vi "AuthService StartLogin.vi"(6 "contextId":T1, 8 "error in":errorcluster, 9 "timeout (ms)":i32=-1, 10 "Request Data":T3, 11 "gRPC ID":T1) -> (0 "error out":errorcluster, 2 "Response Data":T2, 3 "gRPC ID out":T1)   [LabVIEW 2020, in "grpc-auth_client.lvlib"]
uses:
  grpc-auth_client.lvlib
  <vilib>/gRPC/LabVIEW gRPC Library/Shared/grpcId.ctl
  RPC Messages/auth_StartLoginRequest.ctl
  RPC Messages/auth_StartLoginResponse.ctl
  RPC Messages/auth_StartLoginResponse_Flat.ctl
  14035477-4c25-4107-8ed5-d0c4ef420ce5.vi
  <vilib>/gRPC/LabVIEW gRPC Library/Shared/TranslateGrpcError.vi
  <vilib>/gRPC/LabVIEW gRPC Library/Shared/Wait On Occurrence.vi
  <vilib>/gRPC/LabVIEW gRPC Library/Shared/Is Feature Enabled.vi
  <vilib>/gRPC/LabVIEW gRPC Library/Server API/Server/Get Server DLL Path.vi
  <vilib>/Utility/error.llb/Error Cluster From Error Code.vi
  <vilib>/gRPC/LabVIEW gRPC Library/grpc-lvsupport-release.lvlib
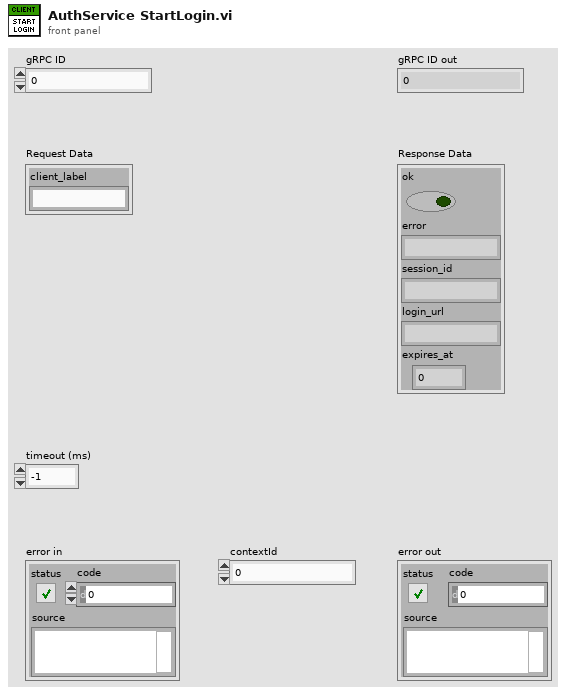
[diagram p1: front panel]
types:
  T1 = typedef "grpc-lvsupport-release.lvlib/grpcId.ctl" = u64
  T2 = typedef "grpc-auth_client.lvlib/auth_StartLoginResponse.ctl" = cluster{"ok":bool, "error":string, "session_id":string, "login_url":string, "expires_at":i64}
  T3 = typedef "grpc-auth_client.lvlib/auth_StartLoginRequest.ctl" = cluster{"client_label":string}
  T4 = typedef "grpc-auth_client.lvlib/auth_StartLoginResponse_Flat.ctl" = cluster{"ok":bool, "error":string, "session_id":string, "login_url":string, "expires_at":i64}
  T5 = typedef "grpc-auth_client.lvlib/auth_StartLoginRequest_Flat.ctl" = cluster{"client_label":string}
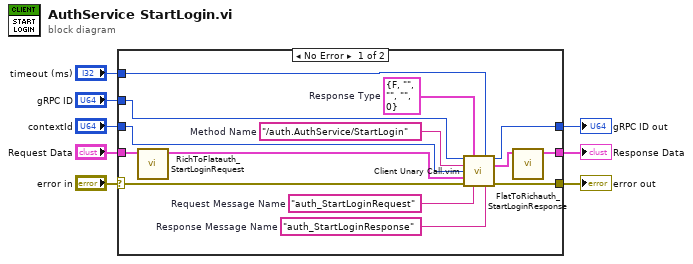
[diagram p0: block diagram]
diagram:
  n1 = case shown="No Error" "error in" {
    selector: "error in" -> [w18 w23]
    tunnel: [w17 w23] -> w7
    tunnel: "gRPC ID" -> [w16 w24]
    tunnel: [w15 w24] -> w5
    tunnel: "Request Data" -> [w12 _]
    tunnel: [w9 _] -> w3
    tunnel: "timeout (ms)" -> [w14 _]
    tunnel: "contextId" -> [w13 _]
    frame No Error {
      w19 = "auth_StartLoginResponse"  # Response Message Name
      w20 = "auth_StartLoginRequest"  # Request Message Name
      w21 = T4 {"ok"=FALSE, "error"="", "session_id"="", "login_url"="", "expires_at"=0}  # Response Type
      w22 = "/auth.AuthService/StartLogin"  # Method Name
      n2 = call "RichToFlatauth_StartLoginRequest.vi"("InputCluster"=w12) -> ("OutputCluster"=w11:T5)  [unwired: 10 in]
      n3 = call "Client Unary Call.vim"("ClientID in"=w16, "Response Type"=w21, "timeout (ms)"=w14, "Method Name"=w22, "contextId"=w13, "Request Data"=w11, "error in"=w18, "Request Message Name"=w20, "Response Message Name"=w19) -> ("ClientID out"=w15:u64, "Response Data"=w10:T4, "error out"=w17:errorcluster)  [unwired: 4 in]
      n4 = call "FlatToRichauth_StartLoginResponse.vi"("InputCluster"=w10) -> ("OutputCluster"=w9:T2)  [unwired: 10 in]
    }
    frame Error {
    }
  }
  "error out" <- w7
  "gRPC ID out" <- w5
  "Response Data" <- w3
